vi "Format_Text_File_Path.vi"(0 "Current Time":timestamp, 5 "Folder Path":path, 11 "Error In":errorcluster) -> (4 "File Path":path, 15 "Error Out":errorcluster)   [LabVIEW 2026, in "Core.lvlib"]
doc: "Generates a formatted text file path using the specified folder path and timestamp information."
uses:
  Core.lvlib
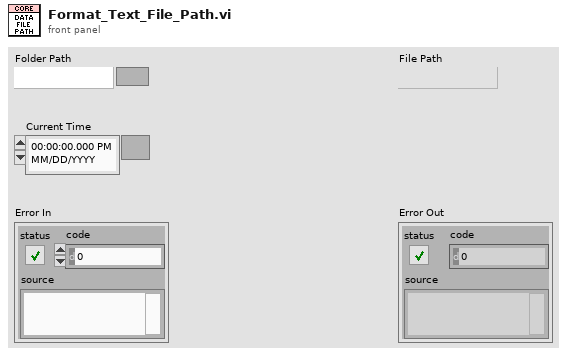
[diagram p1: front panel]
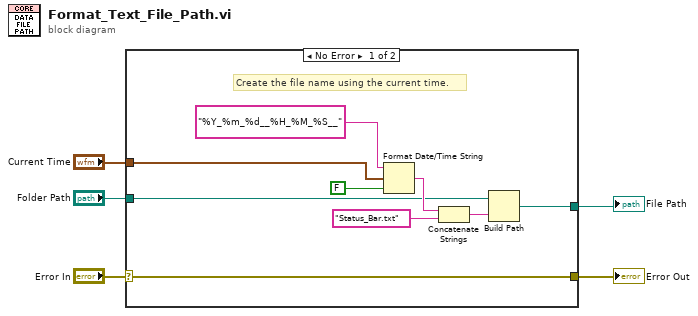
[diagram p0: block diagram]
diagram:
  n1 = case shown="No Error" "Error In" {
    selector: "Error In" -> [w6 w16]
    tunnel: "Current Time" -> [w14 _]
    tunnel: [w8 w15] -> w4
    tunnel: "Folder Path" -> [w7 w15]
    tunnel: [w6 w16] -> w2
    frame No Error {
      # "Create the file name using the current time."
      n2 = Format Date/Time String(time format string (%c)="%Y_%m_%d__%H_%M_%S__", seconds (now)=w14, UTC format=FALSE) -> (date/time string=w10:string)
      n3 = Concatenate Strings(w10, "Status_Bar.txt") -> (w13:string)
      n4 = Build Path(base path=w7, name or relative path=w13) -> (appended path=w8:path)
    }
    frame Error {
    }
  }
  "File Path" <- w4
  "Error Out" <- w2
